vi "LV Config Write.vi"   [LabVIEW 2023]
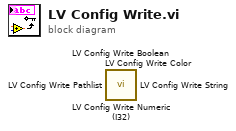
[diagram p0: block diagram]
diagram:
  n1 = call <resource>:"LV Config Write Numeric (I32).vi"() -> ()  [unwired: 7 in, 1 out]
  n2 = call <resource>:"LV Config Write Color.vi"() -> ()  [unwired: 7 in, 1 out]
  n3 = call <resource>:"LV Config Write Pathlist.vi"() -> ()  [unwired: 7 in, 1 out]
  n4 = call <resource>:"LV Config Write String.vi"() -> ()  [unwired: 7 in, 1 out]
  n5 = call <resource>:"LV Config Write Boolean.vi"() -> ()  [unwired: 7 in, 1 out]
